vi "Execute with Default Process Model.vi"() -> ()   [LabVIEW 2020]
uses:
  Execution Options.ctl
  Set Entry Sequence.vi
  Set Sequence File.vi
  Get Result Status.vi
  Engine/Engine.lvclass
  Execution.lvclass
panel:
  in  "Entry Point":string="Single Pass"
  out "Status":string
  in  "SequenceFile Path":path=path "C:/Users/Public/Documents/National Instruments/TestStand 2019 (32-bit)/Examples/Demos/Computer Motherboard Test/LabVIEW/Computer Motherboard Test Sequence.seq"
  # "1."
  # "2."
  # "1. Select the sequence file you'd like to run.\n\n2. Enter the name of the entry point to use in the process model. This is usually 'Test UUTs' or 'Single Pass' for models that ship with TestStand."
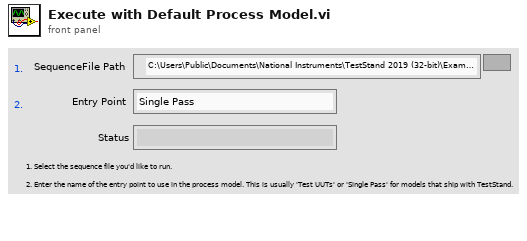
[diagram p1: front panel]
types:
  T1 = typedef "TSS.lvlib/Execution.lvclass/Execution Options.ctl" = cluster{"Use Default Model":bool, "Release Related Sessions":bool}
  T2 = typedef "TSS.lvlib/Engine.lvclass/Session Handle.ctl" = refnum<data-value>
  T3 = typedef "TSS.lvlib/SequenceFile.lvclass/Session Handle.ctl" = refnum<data-value>
  T4 = typedef "TSS.lvlib/Execution.lvclass/Session Handle.ctl" = refnum<data-value>
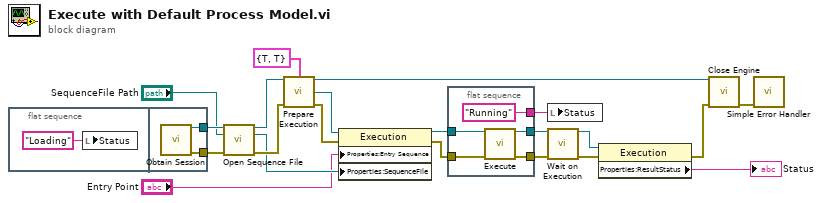
[diagram p0: block diagram]
diagram:
  n1 = flat-sequence {
    tunnel: [w24] -> w21
    tunnel: [w23] -> w15
    frame #0 {
      n2 = local write "Status"("Loading" ("Status")) -> ()
    }
    frame #1 {
      n3 = call "Obtain Session.vi"() -> ("Session Handle"=w24:T2, "error out"=w23:errorcluster)  [unwired: 14 in]
    }
  }
  n4 = call "Open Sequence File.vi"("Engine in"=w21, "File Path"="SequenceFile Path", "error in (no error)"=w15) -> ("Session Handle out"=w8:T2, "SequenceFile"=w6:T3, "error out"=w7:errorcluster)  [unwired: 10 in]
  n5 = call "Prepare Execution.vi"("Session Handle in"=w8, "Options (Default)"=T1 {"Use Default Model"=TRUE, "Release Related Sessions"=TRUE}, "error in (no error)"=w7) -> ("Session Handle out"=w13:T2, "Execution"=w20:T4, "error out"=w14:errorcluster)  [unwired: 10 in]
  n6 = property class="Execution"(reference=w20, error in=w14, "Properties:Entry Sequence"="Entry Point", "Properties:SequenceFile"=w6) -> (reference out=w19:T4, error out=w16:errorcluster)
  n7 = flat-sequence {
    tunnel: w19 -> [w29]
    tunnel: [w28] -> w18
    tunnel: [w27] -> w17
    tunnel: w16 -> [w26]
    tunnel: ["Running" ("Status")] -> w4
    frame #0 {
      n8 = call "Execute.vi"("Session Handle in"=w29, "error in (no error)"=w26) -> ("Session Handle out"=w28:T4, "error out"=w27:errorcluster)  [unwired: 12 in]
    }
  }
  n9 = local write "Status"(w4) -> ()
  n10 = call "Wait on Execution.vi"("Session Handle in"=w18, "error in (no error)"=w17) -> ("Session Handle out"=w12:T4, "error out"=w11:errorcluster)  [unwired: 11 in, 1 out]
  n11 = property class="Execution"(reference=w12, error in=w11) -> (error out=w1:errorcluster, "Properties:ResultStatus"=→"Status":string)  [unwired: 1 out]
  n12 = call "Close Engine.vi"("Session Handle in"=w13, "error in (no error)"=w1) -> ("error out"=w9:errorcluster)  [unwired: 13 in]
  n13 = call <vilib>:"Simple Error Handler.vi"("error in (no error)"=w9) -> ()  [unwired: 4 in, 5 out]
